vi "Untitled 2.vi"() -> ()   [LabVIEW 2026]
uses:
  <vilib>/measure/NI_MABase.lvlib
panel:
  out "signal out 2":waveform(dbl)
  out "signal out":waveform(dbl)
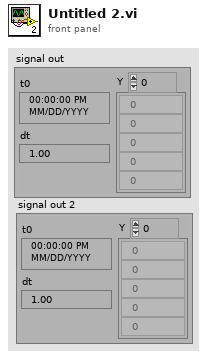
[diagram p1: front panel]
types:
  T1 = enum16{"Sine Wave", "Triangle Wave", "Square Wave", "Sawtooth Wave"}
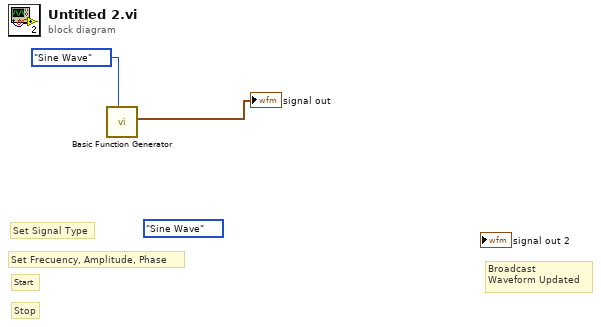
[diagram p0: block diagram]
diagram:
  (unwired) T1."Sine Wave" ("signal type")
  # "Stop"
  # "Start"
  # "Broadcast \nWaveform Updated"
  # "Set Frecuency, Amplitude, Phase"
  # "Set Signal Type"
  n1 = call <vilib>:"Basic Function Generator.vi"("signal type"=T1."Sine Wave") -> ("signal out"=→"signal out":waveform(dbl))  [unwired: 8 in, 2 out]
